vi "PicoScope3000aExampleBlockMSO.vi"() -> ()   [LabVIEW 2010]
uses:
  shared/PicoBuffers.ctl
  <vilib>/Waveform/DWDTOps.llb/DWDT Analog to Digital.vi
  shared/Buffer and Transfer Settings.ctl
  shared/Acquisition Settings.ctl
  PicoScope3000aLib/PicoScope3000aDigitalChannelSettings.ctl
  PicoScope3000aLib/PicoScope3000aAnalogChannelSettings.ctl
panel:
  in  "Trigger Settings":T1={"Trigger Enabled"=FALSE, "Trigger Source"=enum."Channel A", "Trigger Threshold (volts)"=0.0, "Trigger Direction"=2, "Trigger Delay (samples)"=0, "Auto Trigger Time (ms)"=1000} {"Trigger Direction" items=["Above", "Below", "Rising", "Falling", "Rising or Falling"]}
  in  "Channel A Settings":T2={"Enabled"=TRUE, "Coupling"=1, "Range"=6, "Analogue Offset"=0.0, "Bandwidth Limit"=0} {"Bandwidth Limit" items=["Full", "20MHz"]; "Range" items=["10 mV", "20 mV", "50 mV", "100 mV", "200 mV", "500 mV", "1 V", "2 V", "5 V", "10 V", "20 V", "50 V ", "100 V"]; "Coupling" items=["AC", "DC"]}
  in  "Port 0 Settings":T3={"Enabled"=FALSE, "Logic Level"=9830} {"Logic Level" items=["1.5V TTL"=9830, "2.5V CMOS"=16383]}
  out "overflow":i16 format="%010b"
  in  "Apply Settings":bool
  out "USB 3.0 device on non-USB 3.0 Port":bool=TRUE
  out "USB Powered":bool=TRUE
  out "Device Info":T4={"Driver Version"="2.1.104.3324", "USB Version"="2.0", "Hardware"="1", "Variant"="5244A", "Batch and Serial"="CQ178/007", "Cal Date"="11Jun13", "Kernel Version"="1.0", "Digital HW Version"="1", "Analogue HW Version"="1", "MSO"=FALSE, "Number of channels"=2}
  out "error out":errorcluster
  in  "Data file":path=path "PicoScope3000aExampleBlock ChA Data"
  in  "Buffer and Transfer Settings":T5={"startIndex"=0, "Samples"=5000000, "Down Sample Ratio"=1, "Down-Sample Mode"=0} {"Down-Sample Mode" items=["RAW none"=2147483648, "None"=0, "Aggregate"=1, "Decimate"=2, "Average"=4]; "Down Sample Ratio" step=1; "Samples" format="%_6p"}
  in  "Acquisition Settings":T6={"preTriggerSamples"=0, "postTriggerSamples"=5000000, "timebase"=5} {"postTriggerSamples" format="%_6p"; "preTriggerSamples" format="%_6p"}
  out "Properties Panel":T7={"Sample Frequency"=41666668.0, "Sample Rate"=2.4000000209412065e-08, "Max Samples Available"=26843008, "Number of Samples"=0, "Total Capture Time (sec) "=0.0, "Max Total Capture Time Available (sec)"=0.6442322134971619} {"Max Total Capture Time Available (sec)" format="%.3p"; "Sample Frequency" format="%.6p"; "Sample Rate" format="%.3p"; "Max Samples Available" format="%_6p"; "Total Capture Time (sec)" format="%.3p"}
  out "Port 0":digitalwaveform(graph)={"t0"=timestamp(0 s since 1904-01-01), "dt"=8e-09, "Y"={"transitions"=[], "data"=[]}}
  in  "stop":bool
  out "Analog Channels":cluster{i32, sgl, "Data":dbl[]}[](graph)
  in  "Serial Number":string
  in  "Use Serial Number":bool
  in  "error in (no error)":errorcluster
  # "Bit 0 = ChA"
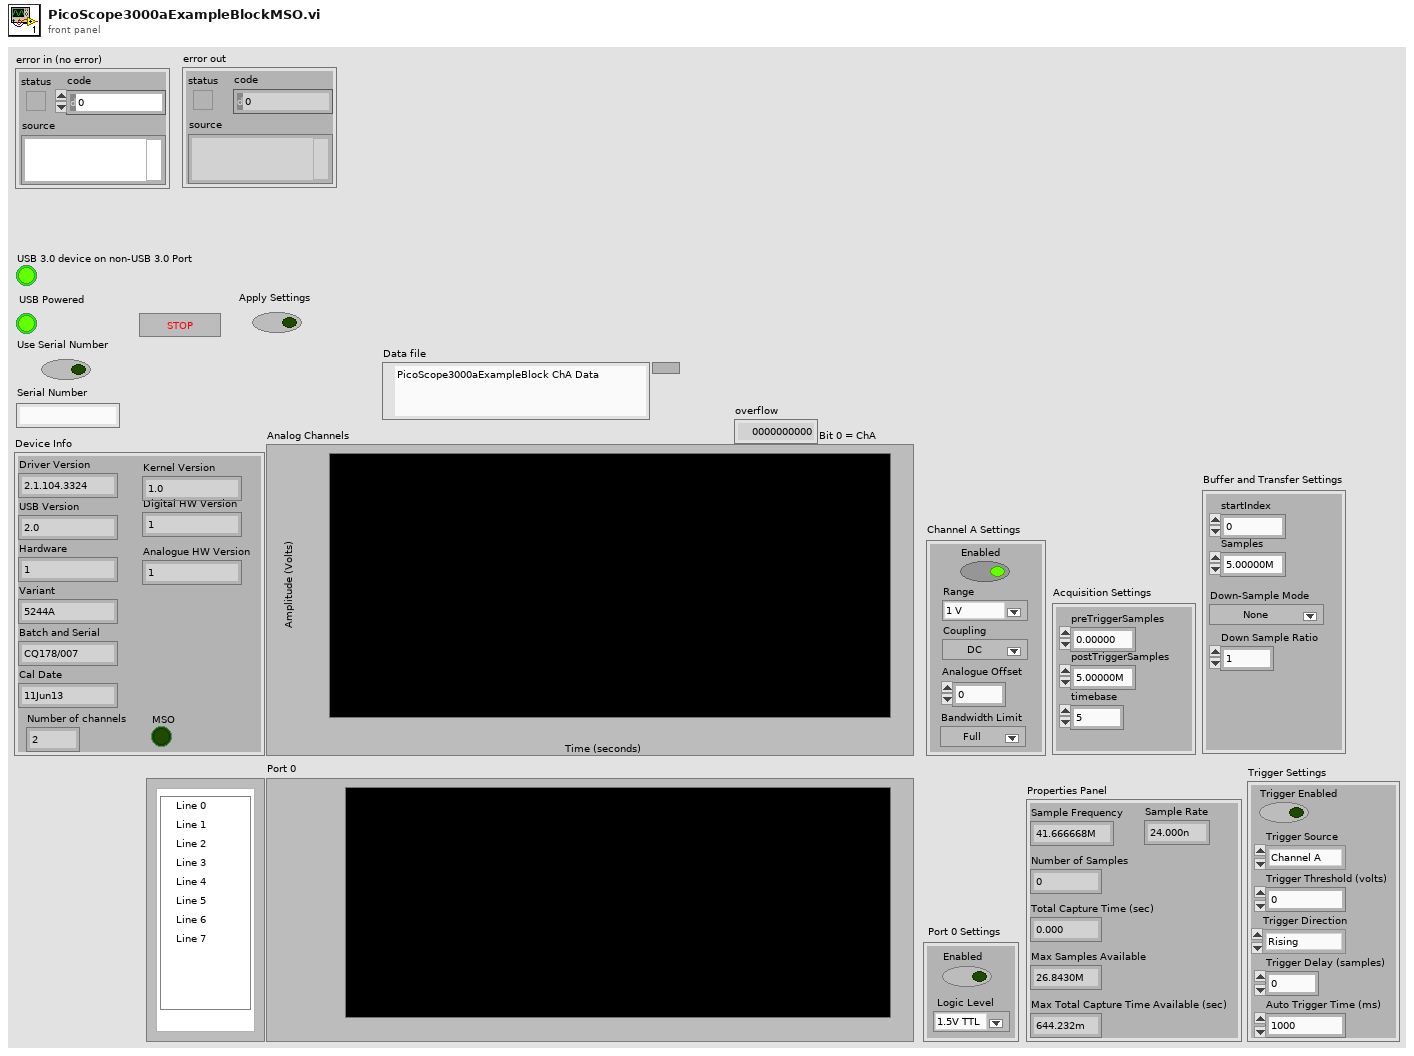
[diagram p1: front panel]
types:
  T1 = cluster{"Trigger Enabled":bool, "Trigger Source":enum32{"Channel A", "Channel B", "Channel C", "Channel D", "Ext."}, "Trigger Threshold (volts)":dbl, "Trigger Direction":u32, "Trigger Delay (samples)":u32, "Auto Trigger Time (ms)":i16}
  T2 = typedef "PicoScope3000aAnalogChannelSettings.ctl" = cluster{"Enabled":bool, "Coupling":u32, "Range":u32, "Analogue Offset":sgl, "Bandwidth Limit":u32}
  T3 = typedef "PicoScope3000aDigitalChannelSettings.ctl" = cluster{"Enabled":bool, "Logic Level":i16}
  T4 = cluster{"Driver Version":string, "USB Version":string, "Hardware":string, "Variant":string, "Batch and Serial":string, "Cal Date":string, "Kernel Version":string, "Digital HW Version":string, "Analogue HW Version":string, "MSO":bool, "Number of channels":i16}
  T5 = typedef "Buffer and Transfer Settings.ctl" = cluster{"startIndex":u64, "Samples":u64, "Down Sample Ratio":u64, "Down-Sample Mode":u32}
  T6 = typedef "Acquisition Settings.ctl" = cluster{"preTriggerSamples":u64, "postTriggerSamples":u64, "timebase":u32}
  T7 = cluster{"Sample Frequency":dbl, "Sample Rate":dbl, "Max Samples Available":u64, "Number of Samples":u64, "Total Capture Time (sec) ":dbl, "Max Total Capture Time Available (sec)":dbl}
  T8 = enum16{"open", "open or create", "create or replace", "create", "open (read-only)"}
  T9 = typedef "PicoBuffers.ctl" = cluster{"Max Buffer Pointers":u64[][][], "Min Buffer Pointers":u64[][][], "StreamingDataInfo":cluster{"Channel":u32, "Down-Sample Mode":u32, "PICO_DATA_TYPE":enum32{"PICO_INT8_T", "PICO_INT16_T", "PICO_INT32_T", "PICO_UINT32_T", "PICO_INT64_T", ""}, "Samples":i32, "bufferIndex":u64, "startIndex":i32, "overflow":i16}[][]}
  T10 = cluster{"Sample Frequency":sgl, "Sample Rate":sgl, "Max Samples Available":i32, "Number of Samples":u32, "Total Capture Time (sec) ":sgl, "Max Total Capture Time Available (sec)":sgl}
  T11 = cluster{"Channel A Buffer":i16[], "Channel B Buffer":i16[], "Channel C Buffer":i16[], "Channel D Buffer":i16[], "Channel E Buffer":i16[], "Channel F Buffer":i16[], "Channel G Buffer":i16[], "Channel H Buffer":i16[], "Port 0 Buffer":i16[], "Port 1 Buffer":i16[]}[]
  T12 = cluster{"Channel A Buffer":i16[], "Channel B Buffer":i16[], "Channel C Buffer":i16[], "Channel D Buffer":i16[], "Channel E Buffer":i16[], "Channel F Buffer":i16[], "Channel G Buffer":i16[], "Channel H Buffer":i16[], "Port 0 Buffer":i16[], "Port 1 Buffer":i16[]}
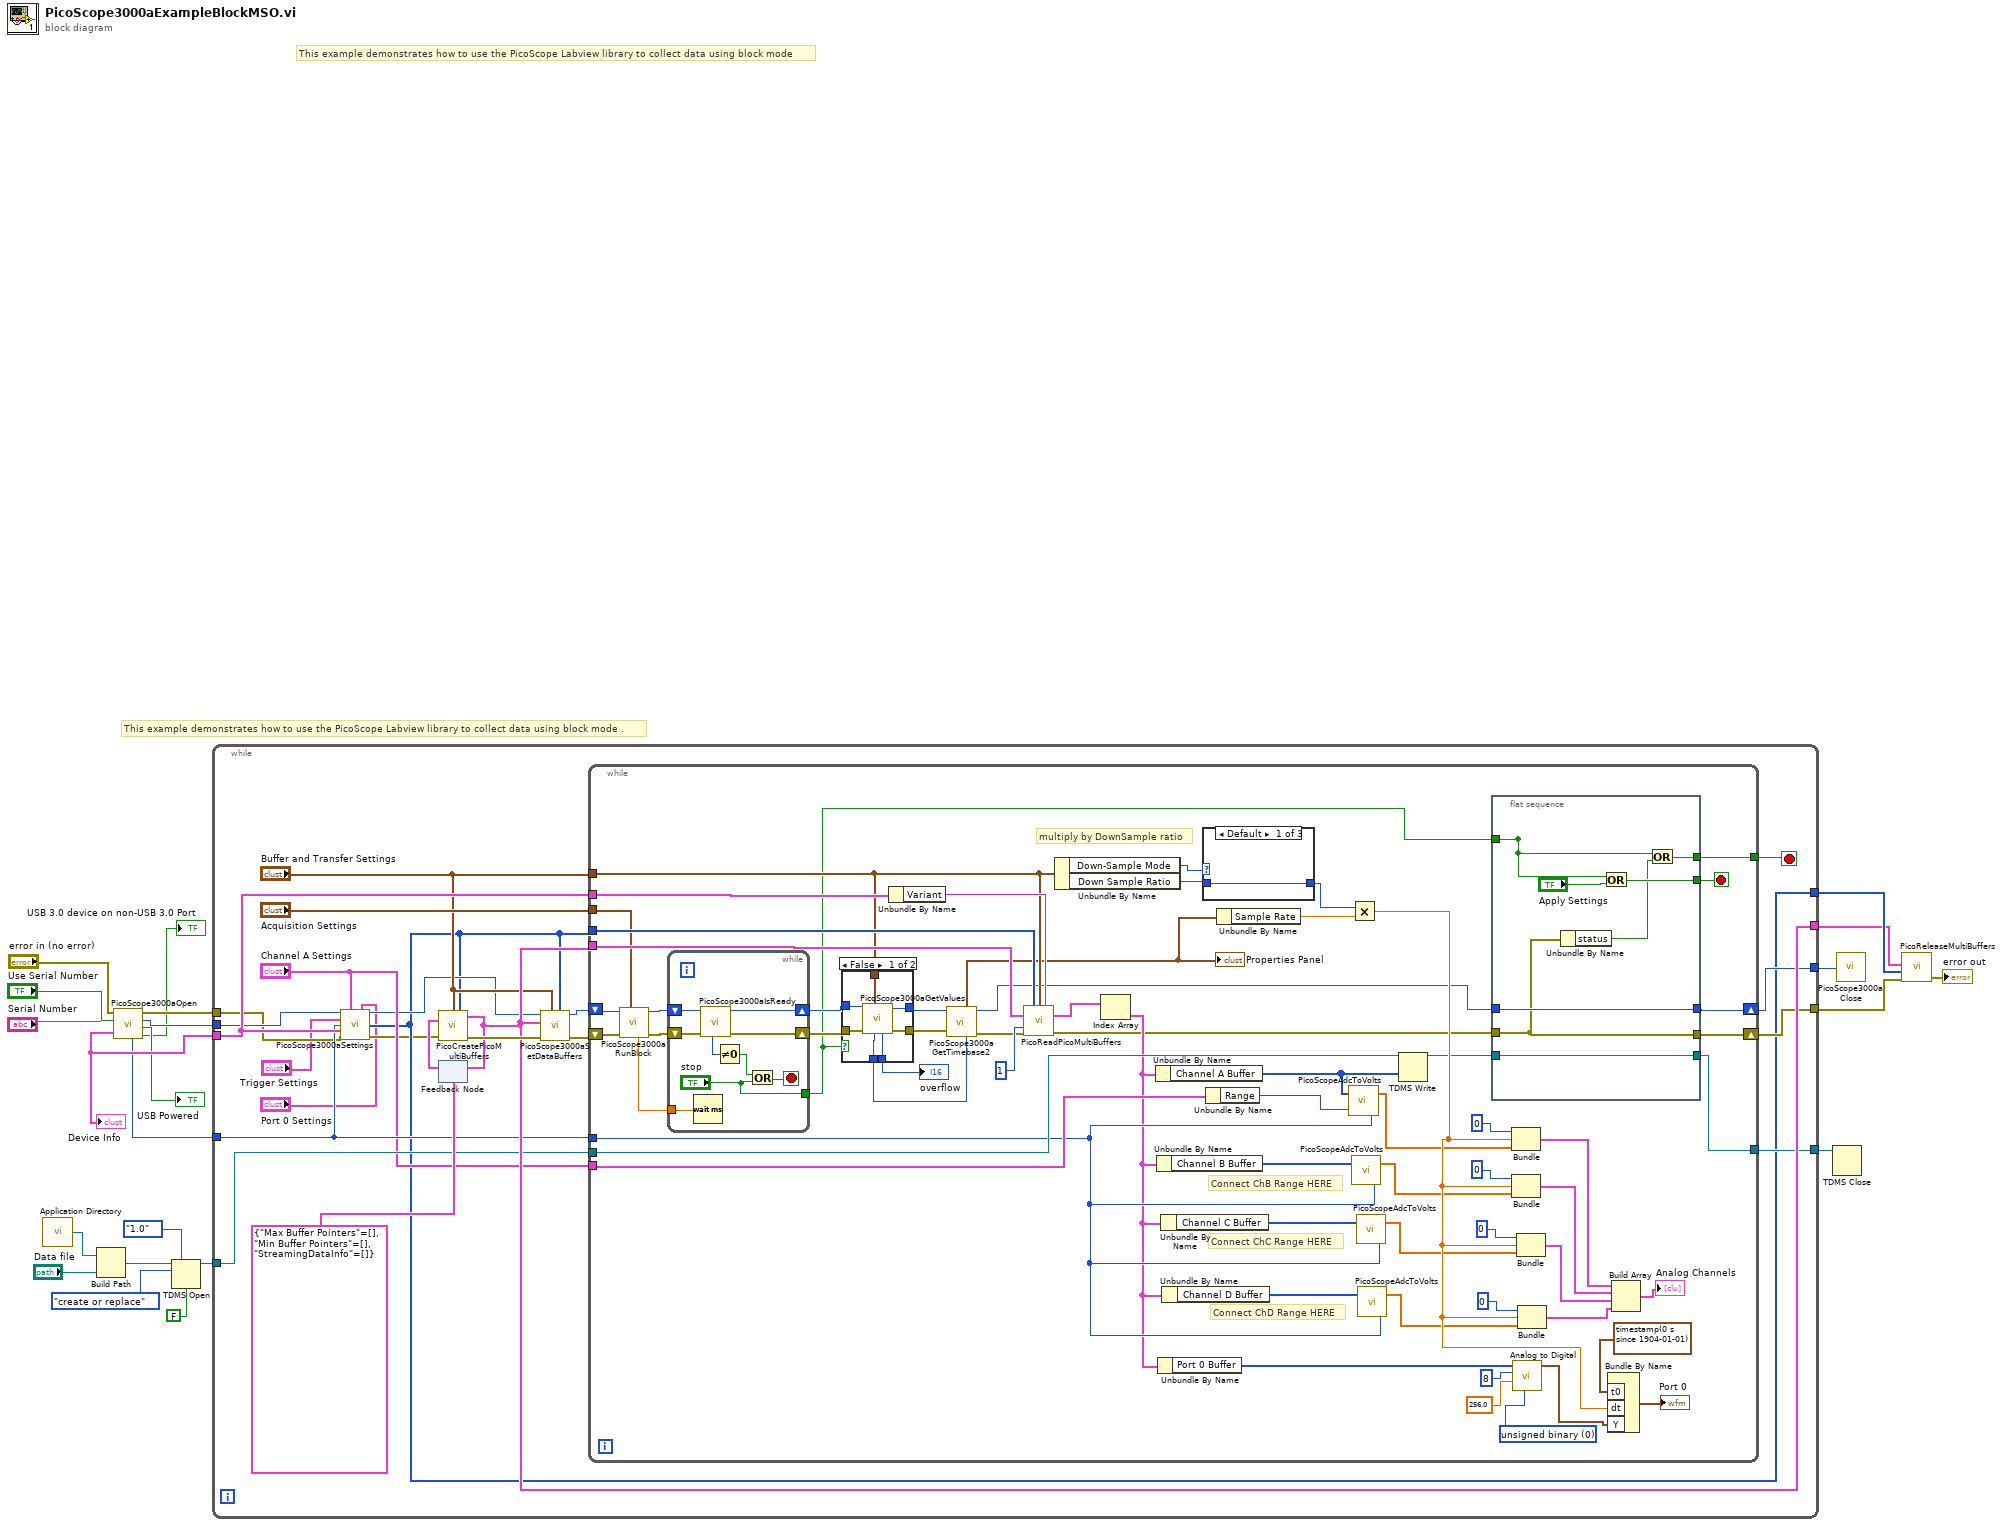
[diagram p0: block diagram]
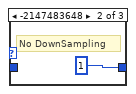
[diagram p3: hidden frame]
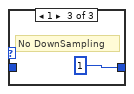
[diagram p4: hidden frame]
diagram:
  # "This example demonstrates how to use the PicoScope Labview library to collect data using block mode ."
  # "This example demonstrates how to use the PicoScope Labview library to collect data using block mode"
  n1 = call <vilib>:"Application Directory.vi"() -> ("Application Directory"=w14:path)
  n2 = Build Path(base path=w14, name or relative path="Data file") -> (appended path=w15:path)
  n3 = call "PicoScope3000aOpen.vi"("Batch/Serial"="Serial Number", "Use Serial number"="Use Serial Number", "error in (no error)"="error in (no error)") -> ("USB 3.0 device on non-USB 3.0 Port"=→"USB 3.0 device on non-USB 3.0 Port":bool, "USB Powered"=→"USB Powered":bool, "handle"=w22:i16, "error out"=w5:errorcluster, "Max ADC value"=w2:i16, "Device Info"=w7:T4)  [unwired: 3 in]
  "Device Info" <- w7
  n4 = TDMS Open(6:FALSE ("disable buffering? (T)"), 7:enum16{"1.0", "2.0"}."1.0" ("file format version (2.0)"), 10:T8."create or replace" ("operation (0:open)"), 11:w15) -> (3:w12:refnum<k34>)  [unwired: 2 in, 1 out]
  n5 = while {
    tunnel: w22 -> [w29]
    tunnel: w2 -> [w31]
    tunnel: [w25] -> w21
    tunnel: [w42] -> w20
    tunnel: [w37] -> w13
    tunnel: w12 -> [w41]
    tunnel: w7 -> [w39]
    tunnel: w5 -> [w28]
    tunnel: [w38] -> w4
    tunnel: [w35] -> w3
    stop <- w36 stop-if-true
    n6 = call "PicoScope3000aSettings.vi"("handle in"=w29, "Channel A Settings"="Channel A Settings", "Port 0 Settings"="Port 0 Settings", "Trigger Settings"="Trigger Settings", "Max_adc"=w31, "Device Info"=w39, "error in"=w28) -> ("handle out"=w26:i16, "Enabled Array"=w25:i16[], "error out"=w24:errorcluster)  [unwired: 6 in]
    n7 = feedback #1(T9 {"Max Buffer Pointers"=[], "Min Buffer Pointers"=[], "StreamingDataInfo"=[]} ("Data Pointers")) -> (w44:T9)
    n8 = call "PicoCreatePicoMultiBuffers.vi"("Buffer and Transfer Settings"="Buffer and Transfer Settings", "enabled array"=w25, "Data Pointers In"=w44, "error in (no error)"=w24) -> ("Data Pointers"=w42:T9, "error out"=w43:errorcluster)  [unwired: 10 in]
    n9 = feedback-in #1(w42) -> ()
    n10 = call "PicoScope3000aSetDataBuffers.vi"("enabled array"=w25, "Buffer and Transfer Settings"="Buffer and Transfer Settings", "error in (no error)"=w43, "Data Pointers In"=w42, "handle in"=w26) -> ("error out"=w34:errorcluster, "handle out"=w33:i16)  [unwired: 5 in]
    n11 = while {
      tunnel: w42 -> [w109]
      tunnel: "Buffer and Transfer Settings" -> [w54]
      tunnel: w25 -> [w100]
      tunnel: "Channel A Settings" -> [w99]
      tunnel: "Acquisition Settings" -> [w98]
      tunnel: w31 -> [w97]
      tunnel: w39 -> [w94]
      tunnel: [w61] -> w36
      shift-right: [w65] -> w38
      shift-left: w34 -> [w55]
      shift-right: [w59] -> w35
      shift-left: w33 -> [w56]
      tunnel: w41 -> [w108]
      tunnel: [w63] -> w37
      stop <- w60 stop-if-true
      w82 = u16 0 items=["unsigned binary", "offset binary", "2's complement"] ("data format (offset binary)")
      # "Connect ChB Range HERE"
      # "Connect ChD Range HERE"
      # "Connect ChC Range HERE"
      # "multiply by DownSample ratio"
      n12 = call "PicoScope3000aRunBlock.vi"("Acquisition Settings"=w98, "error in (no error)"=w55, "handle in"=w56) -> ("error out"=w102:errorcluster, "handle out"=w101:i16, "timeIndisposedMs"=w92:dbl)  [unwired: 5 in, 1 out]
      n13 = while {
        shift-right: [w134] -> w57
        shift-left: w102 -> [w135]
        shift-right: [w133] -> w58
        shift-left: w101 -> [w132]
        tunnel: ["stop"] -> w53
        tunnel: w92 -> [w127]
        stop <- w129 stop-if-true
        n14 = Wait (ms)(milliseconds to wait=w127) -> ()  [unwired: 1 out]
        n15 = call "PicoScope3000aIsReady.vi"("error in (no error)"=w135, "handle in"=w132) -> ("error out"=w134:errorcluster, "handle out"=w133:i16, "ready"=w131:i16)  [unwired: 7 in]
        n16 = Not Equal To 0?(x=w131) -> (x != 0?=w130:bool)
        n17 = Or(x=w130, y="stop") -> (x .or. y?=w129:bool)
      }
      n18 = case shown="False" w53 {
        tunnel: w57 -> [w116 w117]
        tunnel: w58 -> [w115 w118]
        tunnel: [w114 w118] -> w48
        tunnel: [w113 w117] -> w49
        tunnel: w54 -> [w112 _]
        tunnel: [w111 _] -> w52
        tunnel: [w110 _] -> w51
        frame False {
          n19 = call "PicoScope3000aGetValues.vi"("Buffer and Transfer Settings"=w112, "error in (no error)"=w116, "handle in"=w115) -> ("error out"=w113:errorcluster, "handle out"=w114:i16, "overflow"=w111:i16, "noOfSamples"=w110:u64)  [unwired: 5 in]
        }
        frame True {
        }
      }
      "overflow" <- w52
      n20 = Unbundle By Name(w94) -> ("Variant"=w95:string)
      n21 = call "PicoScope3000aGetTimebase2.vi"("Number of Samples"=w51, "error in (no error)"=w49, "handle in"=w48) -> ("error out"=w47:errorcluster, "handle out"=w46:i16, "Properties Panel"=w50:T10)  [unwired: 6 in]
      "Properties Panel" <- w50
      n22 = call "PicoReadPicoMultiBuffers.vi"("enabled array"=w100, "Buffer and Transfer Settings"=w54, "Variant"=w95, "Data Pointers"=w109, "No of Buffers"=1, "error in (no error)"=w47) -> ("MultiBuffers (Max or non-aggregated)"=w107:T11, "error out"=w62:errorcluster)  [unwired: 7 in, 1 out]
      n23 = Unbundle By Name(w54) -> ("Down-Sample Mode"=w105:u32, "Down Sample Ratio"=w106:u64)
      n24 = Index Array(array=w107) -> (element=w66:T12)  [unwired: 1 in]
      n25 = Unbundle By Name(w66) -> ("Channel A Buffer"=w75:i16[])
      n26 = Unbundle By Name(w66) -> ("Channel B Buffer"=w88:i16[])
      n27 = Unbundle By Name(w66) -> ("Port 0 Buffer"=w80:i16[])
      n28 = Unbundle By Name(w66) -> ("Channel C Buffer"=w73:i16[])
      n29 = Unbundle By Name(w66) -> ("Channel D Buffer"=w69:i16[])
      n30 = case shown="Default" w105 {
        tunnel: [w136 u64 1 ("Down Sample Ratio") u64 1 ("Down Sample Ratio")] -> w103
        tunnel: w106 -> [w136 _ _]
        frame Default {
        }
        frame -2147483648 {
          # "No DownSampling"
        }
        frame 1 {
          # "No DownSampling"
        }
      }
      n31 = Unbundle By Name(w99) -> ("Range"=w90:u32)
      n32 = Unbundle By Name(w50) -> ("Sample Rate"=w96:sgl)
      n33 = call "PicoScopeAdcToVolts.vi"("Max_adc"=w97, "Range Index"=w90, "Data"=w75) -> ("Data"=w76:dbl[])
      n34 = Multiply(x=w103, y=w96) -> (x*y=w104:sgl)
      n35 = call "PicoScopeAdcToVolts.vi"("Max_adc"=w97, "Data"=w88) -> ("Data"=w87:dbl[])  [unwired: 1 in]
      n36 = call "PicoScopeAdcToVolts.vi"("Max_adc"=w97, "Data"=w73) -> ("Data"=w72:dbl[])  [unwired: 1 in]
      n37 = call "PicoScopeAdcToVolts.vi"("Max_adc"=w97, "Data"=w69) -> ("Data"=w68:dbl[])  [unwired: 1 in]
      n38 = TDMS Write(0:w108, 9:w75) -> (4:w64:refnum<k34>)  [unwired: 4 in, 3 out]
      n39 = flat-sequence {
        tunnel: [w126] -> w60
        tunnel: [w119] -> _
        tunnel: [w123] -> w61
        tunnel: w46 -> [w122]
        tunnel: [w122] -> w59
        tunnel: w62 -> [w121]
        tunnel: [w121] -> w65
        tunnel: [w120] -> w63
        tunnel: w64 -> [w120]
        tunnel: w53 -> [w119]
        frame #0 {
          n40 = Unbundle By Name(w121) -> ("status"=w124:bool)
          n41 = Or(x=w119, y="Apply Settings") -> (x .or. y?=w126:bool)
          n42 = Or(x=w119, y=w124) -> (x .or. y?=w123:bool)
        }
      }
      n43 = Bundle(0, w104, "Data"=w76) -> (w86:cluster{i32, sgl, "Data":dbl[]})  [unwired: 1 in]
      n44 = Bundle(0, w104, "Data"=w87) -> (w85:cluster{i32, sgl, "Data":dbl[]})  [unwired: 1 in]
      n45 = call-poly <vilib>:"Analog to Digital.vi"("data format (offset binary)"=w82, "full-scale range (pk-pk)"=256.0, "resolution (16 bit)"=8, "analog waveform"=w80) -> ("digital waveform"=w77:digitalwaveform)  [unwired: 4 in, 3 out]
      n46 = Bundle(0, w104, "Data"=w72) -> (w71:cluster{i32, sgl, "Data":dbl[]})  [unwired: 1 in]
      n47 = Bundle(0, w104, "Data"=w68) -> (w67:cluster{i32, sgl, "Data":dbl[]})  [unwired: 1 in]
      n48 = Bundle By Name("t0"=timestamp(0 s since 1904-01-01), "dt"=w104, "Y"=w77) -> (→"Port 0":digitalwaveform)  [unwired: 1 in]
      n49 = Build Array(w86, w85, w71, w67) -> (→"Analog Channels":cluster{i32, sgl, "Data":dbl[]}[])
    }
  }
  n50 = TDMS Close(11:w13) -> ()  [unwired: 1 in, 2 out]
  n51 = call "PicoScope3000aClose.vi"("handle"=w3) -> ()
  n52 = call "PicoReleaseMultiBuffers.vi"("error in (no error)"=w4, "Enabled array"=w21, "Data Pointers"=w20) -> ("error out"=→"error out":errorcluster)  [unwired: 8 in]
